vi "AppendPrivateToken.vi"(11 "DataURL":string) -> (3 "String":string)   [LabVIEW 2017, in "TagDB.lvlib"]
uses:
  TagDB.lvlib
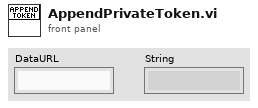
[diagram p1: front panel]
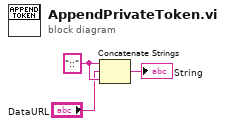
[diagram p0: block diagram]
diagram:
  w3 = "::" ("string")
  n1 = Concatenate Strings(w3, "DataURL", w3) -> (→"String":string)
